vi "Get XML.vi"(8 "error in (no error)":errorcluster, 11 "ToastSource in":refnum<class "ToastSource.lvclass">) -> (0 "error out":errorcluster, 2 "GetContent":string, 3 "ToastSource out":refnum<class "ToastSource.lvclass">)   [LabVIEW 2026, in "ToastNotification.lvlib" / "ToastSource.lvclass"]
doc: "Dynamic XML export operation for a concrete ToastSource. Skipped on incoming error. The base method returns an empty GetContent string and passes the source and error through; it does not serialize content. Override it to return toast XML as a LabVIEW string without displaying a notification or transferring native references."
uses:
  ToastSource.lvclass
  ToastSource.lvclass/ToastSource.ctl
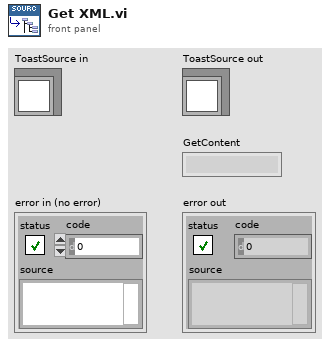
[diagram p1: front panel]
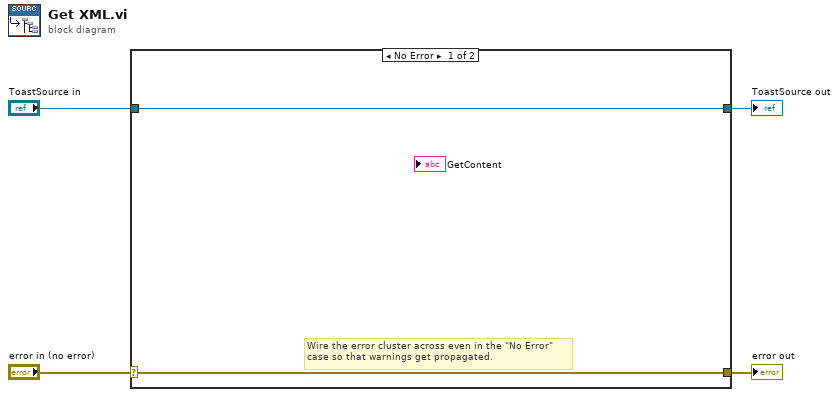
[diagram p0: block diagram]
diagram:
  n1 = case shown="No Error" "error in (no error)" {
    selector: "error in (no error)" -> [w5 w8]
    tunnel: [w5 w8] -> w3
    tunnel: [w6 w7] -> w1
    tunnel: "ToastSource in" -> [w6 w7]
    frame No Error {
      # "Wire the error cluster across even in the \"No Error\"\ncase so that warnings get propagated."
    }
    frame Error {
    }
  }
  "error out" <- w3
  "ToastSource out" <- w1
